vi "VM Spy - build context list shortcut menu.vi"(9 "Coords":T1, 10 "MenuRef":refnum<k9>, 11 "CtlRef":refnum<vi>) -> (0 "Discard menu":bool, 3 "Value changed":bool)   [LabVIEW 2021]
doc: "::: CalcExpress Toolkit :::\nCopyright (c) 2000-2026 Konstantin Shifershteyn. All rights reserved."
uses:
  <vilib>/Utility/miscctls.llb/LVPoint32TypeDef.ctl
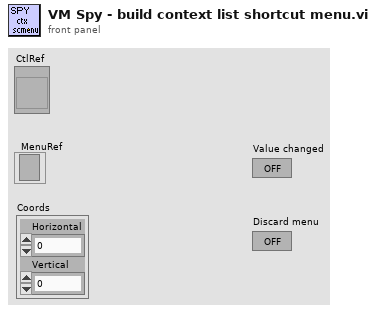
[diagram p1: front panel]
types:
  T1 = typedef "LVPoint32TypeDef.ctl" = cluster{"Horizontal":i32, "Vertical":i32}
  T2 = typedef "LVRowAndColumnTypeDef.ctl" = cluster{"Row":i32, "Column":i32}
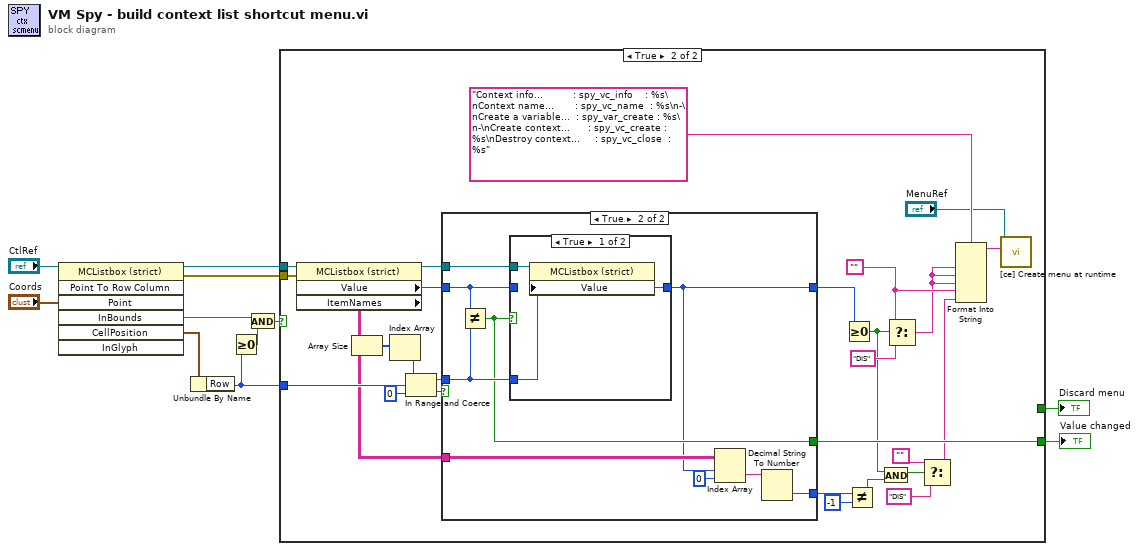
[diagram p0: block diagram]
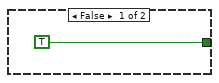
[diagram p2: hidden frame]
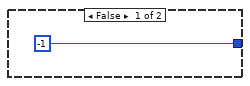
[diagram p3: hidden frame]
diagram:
  n1 = invoke class="MCListbox (strict)" method="Point To Row Column"(reference="CtlRef", "Point"="Coords") -> (reference out=w9:refnum<vi>, error out=w8:errorcluster, "InBounds"=w6:bool, "CellPosition"=w3:T2)  [unwired: 5 in, 3 out]
  n2 = Unbundle By Name(w3) -> ("Row"=w2:i32)
  n3 = Greater Or Equal To 0?(x=w2) -> (x >= 0?=w4:bool)
  n4 = And(x=w6, y=w4) -> (x .and. y?=w5:bool)
  n5 = case shown="True" w5 {
    tunnel: w9 -> [_ w39]
    tunnel: w8 -> [_ w38]
    tunnel: [TRUE _] -> w7
    tunnel: w2 -> [_ w27]
    tunnel: [_ w23] -> w1
    frame False {
    }
    frame True {
      w24 = ""
      n6 = property class="MCListbox (strict)"(reference=w39, error in=w38) -> (reference out=w31:refnum<vi>, "Value"=w32:i32, "ItemNames"=w21:string[][])  [unwired: 1 out]
      n7 = Array Size(array=w21) -> (size(s)=w37:i32[])
      n8 = Index Array(array=w37) -> (element=w36:i32)  [unwired: 1 in]
      n9 = In Range and Coerce(upper limit=w36, x=w27, lower limit=0) -> (coerced(x)=w33:i32, In Range?=w34:bool)
      n10 = case shown="True" w34 {
        tunnel: w33 -> [_ w47]
        tunnel: w32 -> [_ w48]
        tunnel: w31 -> [_ w49]
        tunnel: [-1 ("lower limit") w44] -> w26
        tunnel: [_ w46] -> w23
        tunnel: w21 -> [_ w45]
        tunnel: [_ w41] -> w20
        frame False {
        }
        frame True {
          n11 = Not Equal?(x=w48, y=w47) -> (x != y?=w46:bool)
          n12 = case shown="True" w46 {
            tunnel: w49 -> [w51 _]
            tunnel: [w50 w52] -> w44
            tunnel: w48 -> [_ w52]
            tunnel: w47 -> [w50 _]
            frame True {
              n13 = property class="MCListbox (strict)"(reference=w51, "Value"=w50) -> ()  [unwired: 1 in, 2 out]
            }
            frame False {
            }
          }
          n14 = Index Array(array=w45, index (row)=w44, index (col)=0 ("disabled index (col)")) -> (element=w42:string)
          n15 = Decimal String To Number(string=w42) -> (number=w41:i32)  [unwired: 2 in, 1 out]
        }
      }
      n16 = Greater Or Equal To 0?(x=w26) -> (x >= 0?=w14:bool)
      n17 = Not Equal?(x=w20, y=-1) -> (x != y?=w15:bool)
      n18 = And(x=w14, y=w15) -> (x .and. y?=w17:bool)
      n19 = Select(t=w24, s=w14, f="DIS") -> (s? t:f=w22:string)
      n20 = Select(t="", s=w17, f="DIS") -> (s? t:f=w13:string)
      n21 = Format Into String(format string="Context info...          : spy_vc_info    : %s\nContext name...       : spy_vc_name  : %s\n-\nCreate a variable...  : spy_var_create : %s\n-\nCreate context...      : spy_vc_create : %s\nDestroy context...     : spy_vc_close  : %s", w22, w22, w22, w24, w13) -> (resulting string=w28:string)  [unwired: 2 in, 1 out]
      n22 = call "[ce] Create menu at runtime.vi"("menu descriptor"=w28, "menu"="MenuRef") -> ()  [unwired: 8 in, 2 out]
    }
  }
  "Discard menu" <- w7
  "Value changed" <- w1
